vi "Test Generate Mock Class Implements Mocked Interface.vi"(8 "error in (no error)":errorcluster, 11 "Test Case In":refnum<class "_Mock Class Generator Test.lvclass">) -> (0 "error out":errorcluster, 3 "Test Case Out":refnum<class "_Mock Class Generator Test.lvclass">)   [LabVIEW 2020, in "_Mock Class Generator Test.lvclass"]
uses:
  _Mock Class Generator Test.lvclass
  C:/Program Files (x86)/National Instruments/LabVIEW 2020/vi.lib/Astemes/LUnit/Test Case.lvclass
  <vilib>/Astemes/LUnit/Test Case.lvclass/Test Case.ctl
  d61b9b24-4b0f-44ef-a9bb-4996cb077d5f.vi
  <vilib>/Astemes/LUnit/Append Pass Result.vi
  <vilib>/Astemes/LUnit/Append Fail Result.vi
  <vilib>/Astemes/LUnit/Describe Comparison.vi
  <vilib>/Astemes/LUnit/Compare Variants.vi
  <vilib>/Astemes/LUnit/Run In UI.vi
  <vilib>/Utility/error.llb/Clear Errors.vi
  <vilib>/Astemes/LUnit/Describe Variant.vi
  _Mock Class Generator Test.lvclass/_Mock Class Generator Test.ctl
  source/Scripting/Mock Class Generator/Mock Class Generator.lvclass
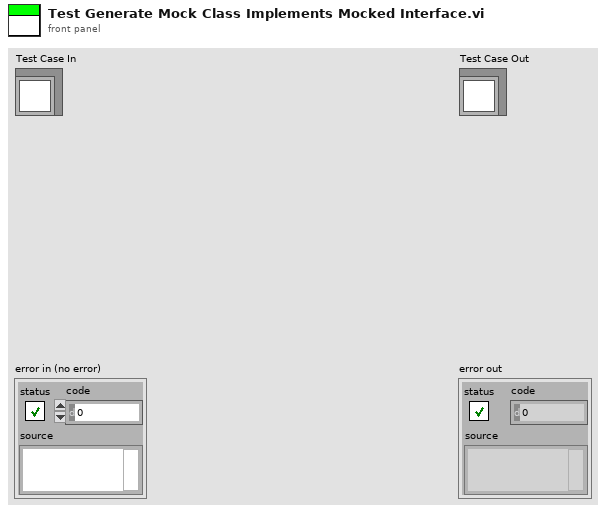
[diagram p1: front panel]
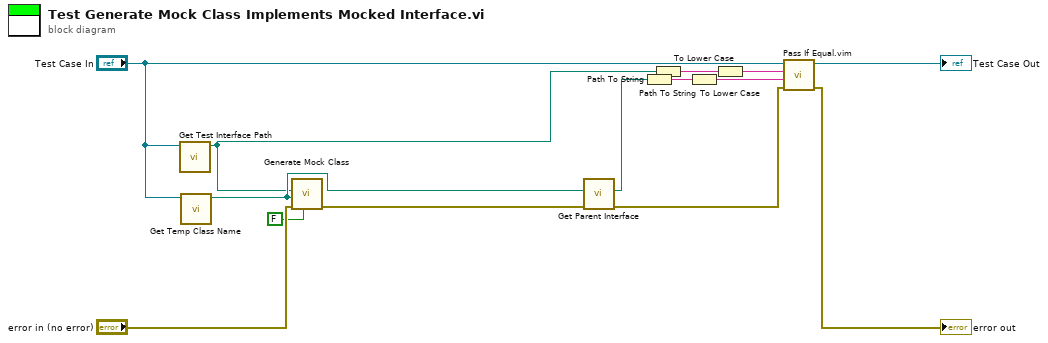
[diagram p0: block diagram]
diagram:
  n1 = call "Get Test Interface Path.vi"("Mock Class Generator Test in"="Test Case In") -> ("Test Class Path"=w5:path)  [unwired: 10 in]
  n2 = call "Get Temp Class Name.vi"("Mock Class Generator Test in"="Test Case In") -> ("Test Class Path"=w11:path)  [unwired: 10 in]
  n3 = call "Generate Mock Class.vi"("Add to lvproj?"=FALSE, "error in (no error)"="error in (no error)", "Destination Class Path"=w11, "Source Class Path"=w5) -> ("error out"=w10:errorcluster)  [unwired: 6 in, 1 out]
  n4 = call "Get Parent Interface.vi"("error in (no error)"=w10, "Test Class Path"=w11) -> ("error out"=w9:errorcluster, "Path"=w8:path)  [unwired: 8 in]
  n5 = Path To String(path=w8) -> (string=w3:string)
  n6 = Path To String(path=w5) -> (string=w2:string)
  n7 = To Lower Case(string=w3) -> (all lower case string=w4:string)
  n8 = To Lower Case(string=w2) -> (all lower case string=w1:string)
  n9 = call "Pass If Equal.vim"("error in (no error)"=w9, "Actual"=w4, "Expected"=w1, "LUnit Test Case In"="Test Case In") -> ("error out"=→"error out":errorcluster, "LUnit Test Case Out"=→"Test Case Out":refnum<class "_Mock Class Generator Test.lvclass">)  [unwired: 6 in]
